vi "ACQ_SharedState_Transport_Auto.vi"() -> ()   [LabVIEW 2012]
panel:
  out "Telemetry packet flatten error":errorcluster caption="sortie d'erreur"
  out "Telemetry stop queue dequeue error":errorcluster caption="sortie d'erreur"
  out "Telemetry stop queue obtain error":errorcluster caption="sortie d'erreur"
  out "Queue cleanup error 2":errorcluster caption="sortie d'erreur"
  out "Queue cleanup error":errorcluster caption="sortie d'erreur"
  in  "packet":variant
  in  "Stop telemetry transport":bool
  out "Ack length in range (required)":bool
  out "Telemetry transport error only":errorcluster caption="sortie d'erreur"
  out "Ack JSON (raw; not validated)":string
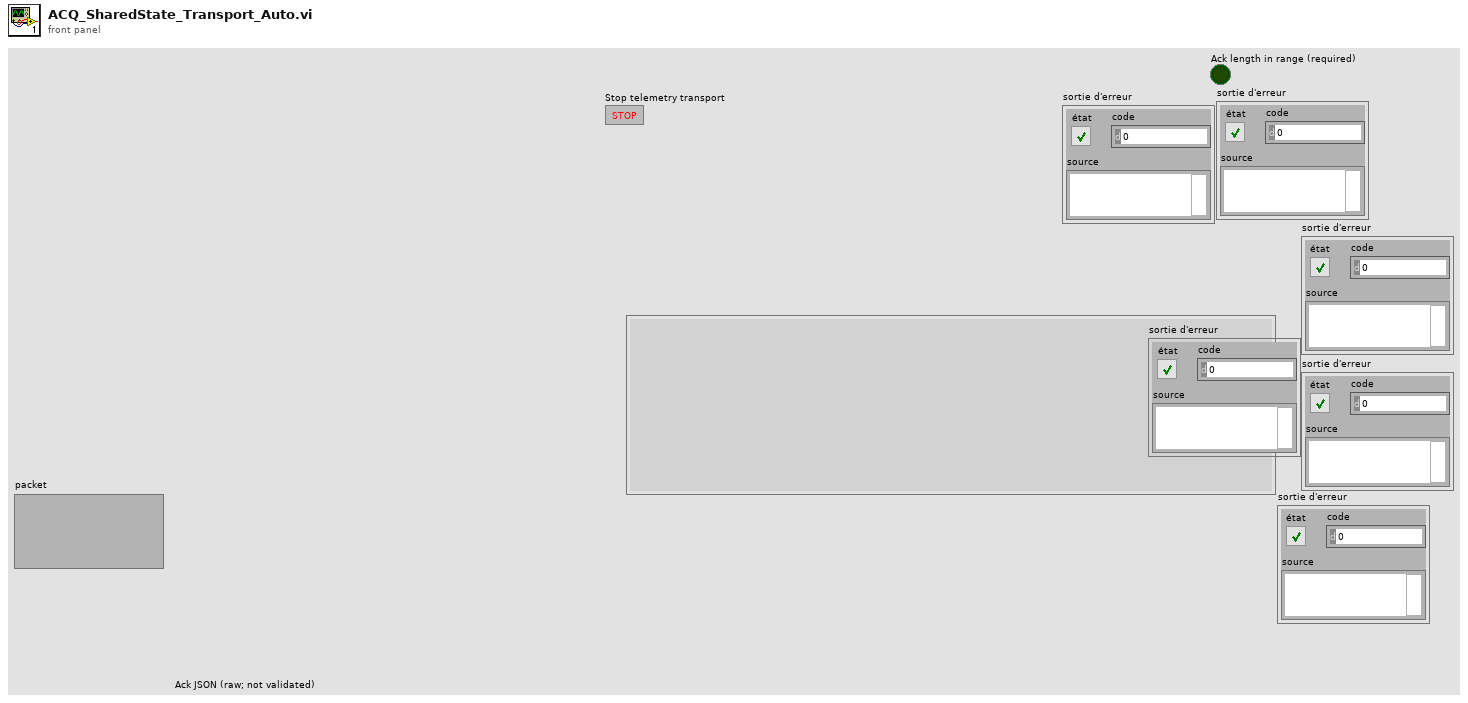
[diagram p1: front panel]
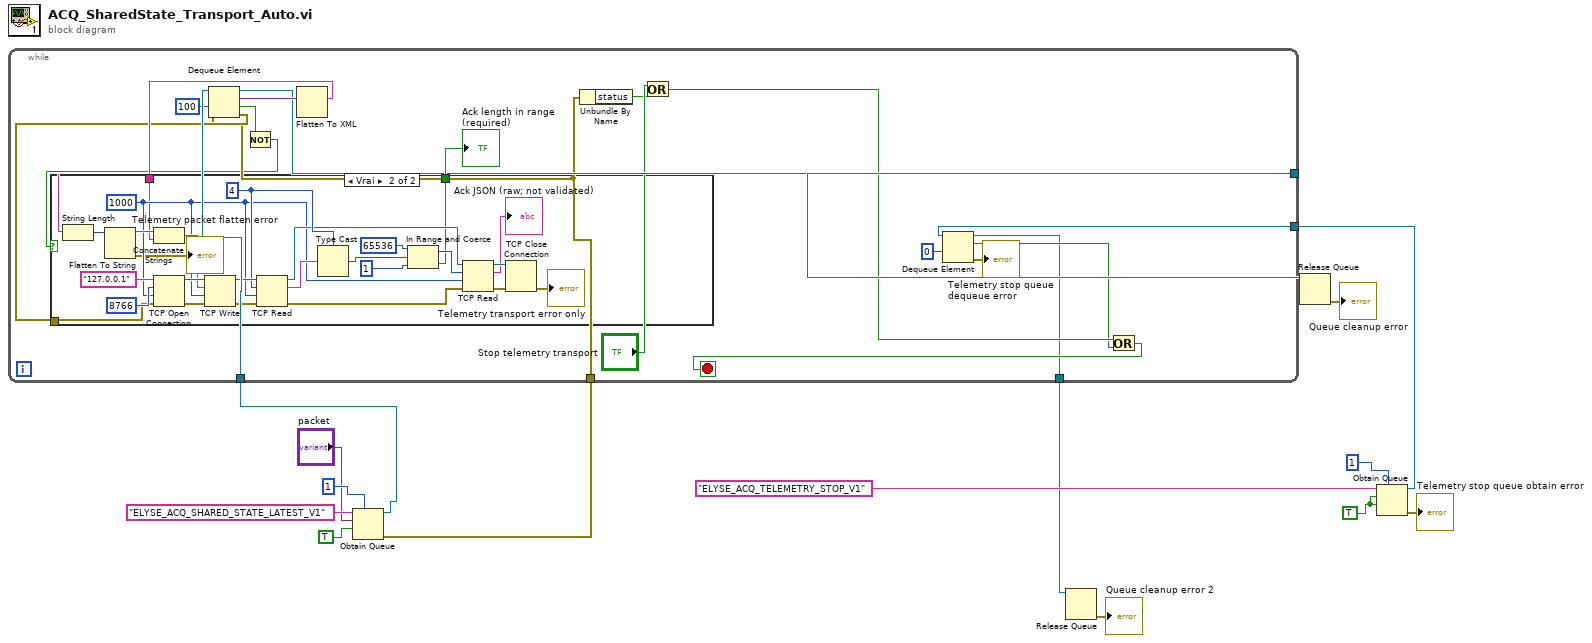
[diagram p0: block diagram]
diagram:
  w5 = TRUE ("créer si introuvable ? (V)")
  n1 = Obtain Queue(max queue size (-1, unlimited)=1 ("taille max de la file d'attente (-1, non limitée)"), name (unnamed)="ELYSE_ACQ_SHARED_STATE_LATEST_V1" ("nom (aucun)"), element data type="packet", create if not found? (T)=TRUE ("créer si introuvable ? (V)")) -> (queue out=w11:refnum<queue>, error out=w10:errorcluster)  [unwired: 1 in, 1 out]
  n2 = Obtain Queue(max queue size (-1, unlimited)=1 ("taille max de la file d'attente (-1, non limitée)"), name (unnamed)="ELYSE_ACQ_TELEMETRY_STOP_V1" ("nom (aucun)"), element data type=w5, create if not found? (T)=w5) -> (queue out=w4:refnum<queue>, error out=→"Telemetry stop queue obtain error":errorcluster)  [unwired: 1 in, 1 out]
  n3 = while {
    tunnel: w11 -> [w33]
    tunnel: w10 -> [w27]
    tunnel: [w28] -> w9
    tunnel: w4 -> [w21]
    tunnel: [w17] -> w2
    stop <- w18 stop-if-true
    n4 = Dequeue Element(queue=w33, timeout in ms (-1)=100 ("timeout en ms (-1)"), error in (no error)=w27) -> (queue out=w28:refnum<queue>, element=w31:variant, timed out?=w24:bool, error out=w29:errorcluster)
    n5 = Not(x=w24) -> (.not. x?=w23:bool)
    n6 = Flatten To XML(anything=w31) -> (xml string=w30:string)
    n7 = case shown="Vrai" w23 {
      tunnel: [_ w38] -> w34
      tunnel: w30 -> [_ w37]
      tunnel: w29 -> [_ w36]
      frame False {
      }
      frame True {
        w41 = 1000 ("timeout en ms (60000)")
        w51 = 4 ("octets à lire")
        n8 = String Length(string=w37) -> (length=w56:i32)
        n9 = Flatten To String(anything=w56) -> (data string=w55:string, error out=→"Telemetry packet flatten error":errorcluster)  [unwired: 3 in, 1 out]
        n10 = Concatenate Strings(w55, w37) -> (w54:string)
        n11 = TCP Open Connection(address="127.0.0.1" ("adresse"), remote port or service name=u16 8766 ("port distant ou nom du service"), timeout ms (60000)=w41, error in (no error)=w36) -> (connection ID=w58:refnum<k5>, error out=w57:errorcluster)  [unwired: 1 in]
        n12 = TCP Write(connection ID=w58, data in=w54, error in (no error)=w57, 9:w41) -> (connection ID out=w53:refnum<k5>, error out=w52:errorcluster)  [unwired: 1 out]
        n13 = TCP Read(connection ID=w53, bytes to read=w51, error in (no error)=w52, 9:w41) -> (connection ID out=w49:refnum<k5>, data out=w50:string, error out=w48:errorcluster)  [unwired: 1 in]
        n14 = Type Cast(type=w51, x=w50) -> (*(type *) &x=w47:i32)
        n15 = In Range and Coerce(upper limit=65536 ("limite supérieure"), x=w47, lower limit=1 ("limite inférieure")) -> (coerced(x)=w44:i32, In Range?=w38:bool)
        n16 = TCP Read(connection ID=w49, bytes to read=w44, error in (no error)=w48, 9:w41) -> (connection ID out=w43:refnum<k5>, data out=→"Ack JSON (raw; not validated)":string, error out=w42:errorcluster)  [unwired: 1 in]
        n17 = TCP Close Connection(connection ID=w43, error in (no error)=w42) -> (error out=→"Telemetry transport error only":errorcluster)  [unwired: 1 in, 1 out]
      }
    }
    "Ack length in range (required)" <- w34
    n18 = Unbundle By Name(w27) -> ("status"=w25:bool)
    n19 = Or(x="Stop telemetry transport", y=w25) -> (x .or. y?=w20:bool)
    n20 = Dequeue Element(queue=w21, timeout in ms (-1)=0 ("timeout en ms (-1)")) -> (queue out=w17:refnum<queue>, element=w19:bool, error out=→"Telemetry stop queue dequeue error":errorcluster)  [unwired: 1 in, 1 out]
    n21 = Or(x=w20, y=w19) -> (x .or. y?=w18:bool)
  }
  n22 = Release Queue(queue=w2) -> (error out=→"Queue cleanup error 2":errorcluster)  [unwired: 2 in, 2 out]
  n23 = Release Queue(queue=w9) -> (error out=→"Queue cleanup error":errorcluster)  [unwired: 2 in, 2 out]
